vi "base color selection_N.vi"(10 "path":string="000.csv", 11 "Sample Sequence":string="GATGATGATGATGATGAT") -> (2 "element":string, 3 "Base All Composition":T1(array[cluster]))   [LabVIEW 2018]
panel:
  out "error out":errorcluster
  in  "error in":errorcluster
  out "Base C":string[](array[string])
  out "Base Composition":string[](array[string])
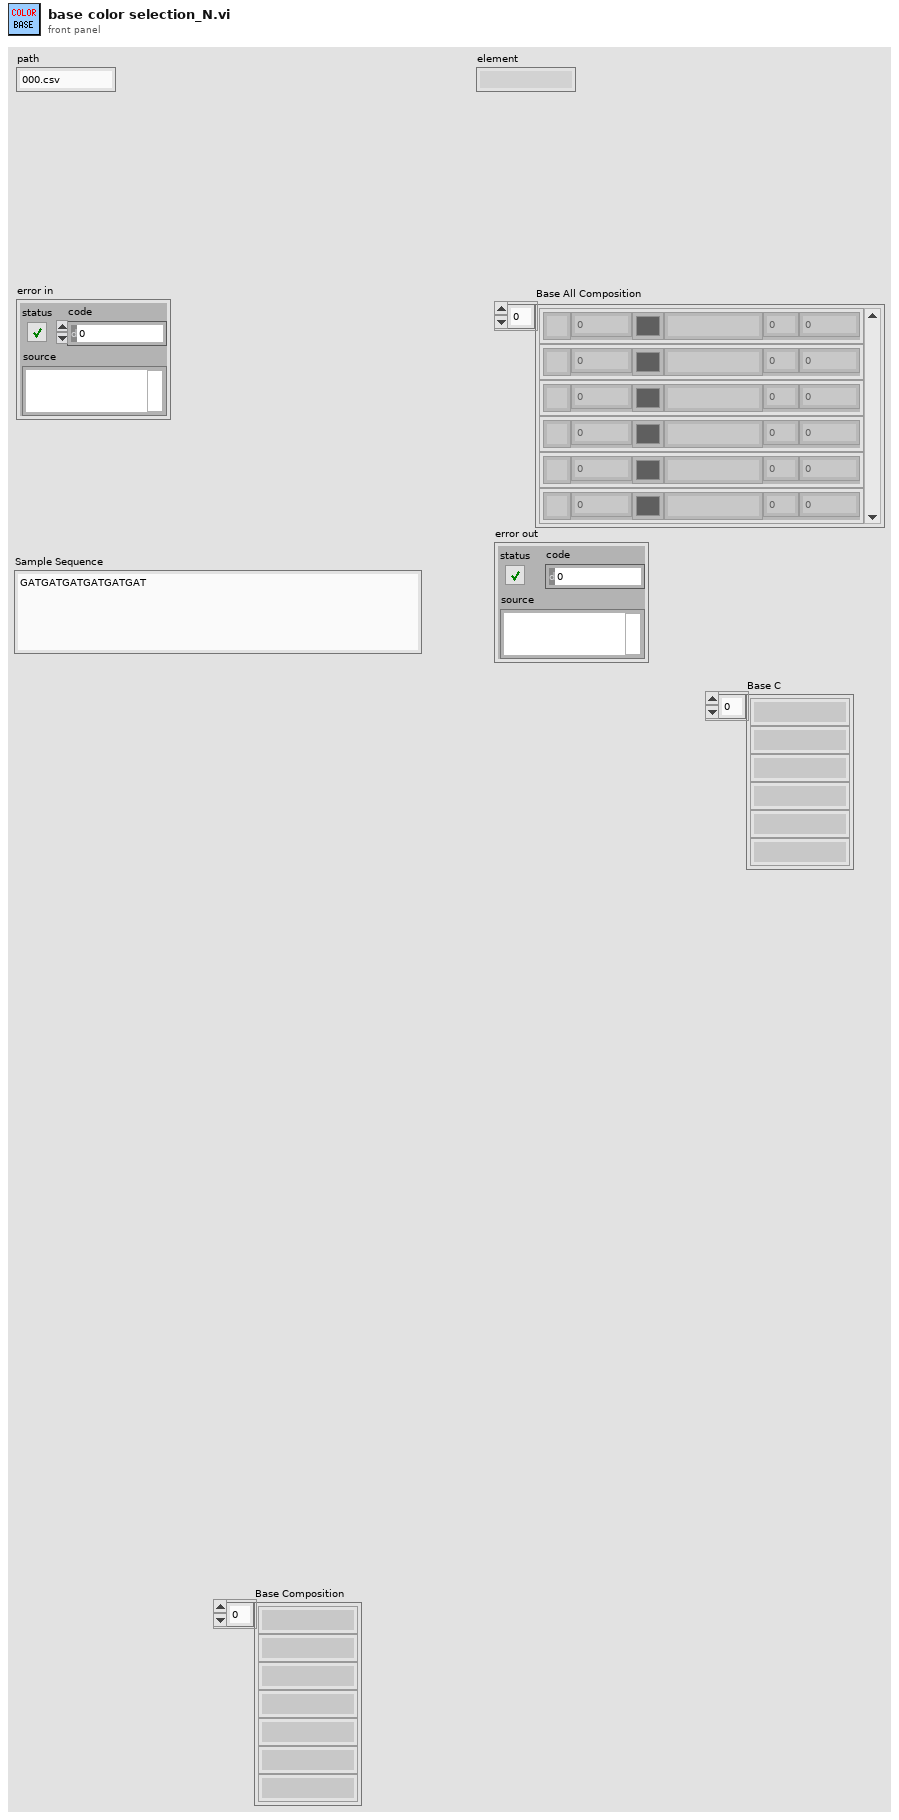
[diagram p1: front panel]
types:
  T1 = cluster{"Name":string, "Value":dbl, "Color":u32, "Name 2":string, "Value 2":dbl, "Value 3":dbl}[]
  T2 = cluster{"Name":string, "Value":dbl, "Color":u32, "Name 2":string, "Value 2":dbl, "Value 3":dbl}
  T3 = cluster{"Base Species IDX":i32, "Item":cluster{"Name":string, "Value":dbl, "Color":u32, "Name 2":string, "Value 2":dbl, "Value 3":dbl}}
  T4 = cluster{"Base Species IDX":i32, "Item":cluster{"Name":string, "Value":dbl, "Color":u32, "Name 2":string, "Value 2":dbl, "Value 3":dbl}}[]
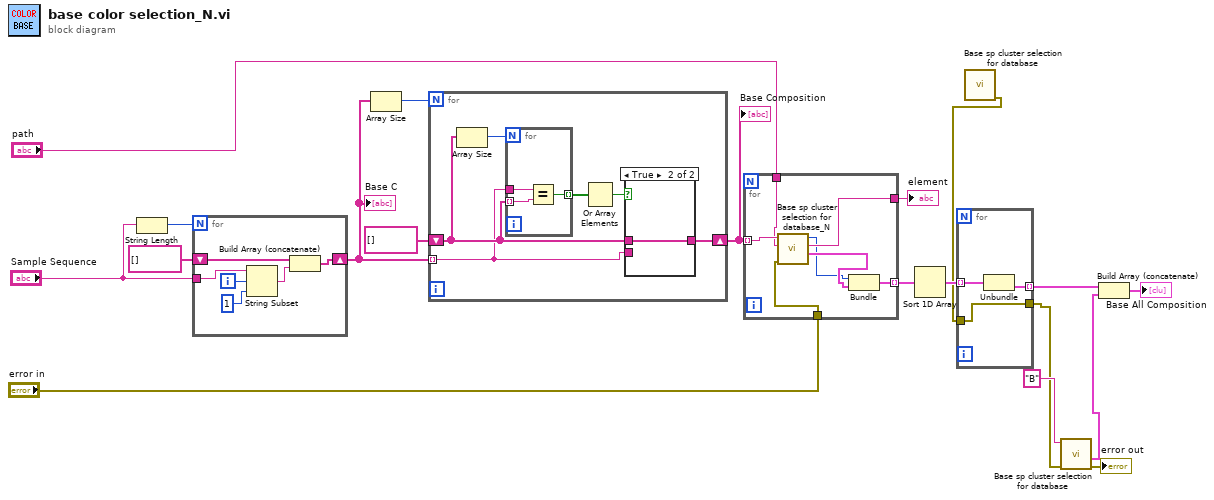
[diagram p0: block diagram]
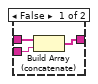
[diagram p2: hidden frame]
diagram:
  n1 = String Length(string="Sample Sequence") -> (length=w19:i32)
  n2 = for {
    N: w19 -> [_]
    tunnel: "Sample Sequence" -> [w23]
    shift-right: [w22] -> w14
    shift-left: string[] [] -> [w21]
    i -> [w24]
    n3 = String Subset(string=w23, offset (0)=w24, length (rest)=1 ("長さ（残り）")) -> (substring=w20:string)
    n4 = Build Array (concatenate)(w21, w20) -> (w22:string[])
  }
  "Base C" <- w14
  n5 = Array Size(array=w14) -> (size(s)=w16:i32)
  n6 = for {
    N: w16 -> [_]
    tunnel: w14 -> [w28] mode=indexing
    shift-right: [w31] -> w11
    shift-left: string[] [] -> [w29]
    n7 = Array Size(array=w29) -> (size(s)=w30:i32)
    n8 = for {
      N: w30 -> [_]
      tunnel: w29 -> [w38] mode=indexing
      tunnel: w28 -> [w37]
      tunnel: [w36] -> w27 mode=indexing
      n9 = Equal?(x=w37, y=w38) -> (x = y?=w36:bool)
    }
    n10 = Or Array Elements(Boolean array=w27) -> (logical OR=w26:bool)
    n11 = case shown="True" w26 {
      tunnel: [w34 w35] -> w31
      tunnel: w29 -> [w33 w35]
      tunnel: w28 -> [w32 _]
      frame False {
        n12 = Build Array (concatenate)(w33, w32) -> (w34:string[])
      }
      frame True {
      }
    }
  }
  "Base Composition" <- w11
  n13 = for {
    tunnel: w11 -> [w43] mode=indexing
    tunnel: [w45] -> w13 mode=indexing
    tunnel: "error in" -> [w44]
    tunnel: [w41] -> w3
    tunnel: "path" -> [w39]
    n14 = call "Base sp cluster selection for database_N.vi"("error in"=w44, "path"=w39, "Base"=w43) -> ("Item"=w42:T2, "element"=w41:string, "Base Species IDX"=w40:i32)  [unwired: 5 in, 1 out]
    n15 = Bundle("Base Species IDX"=w40, "Item"=w42) -> (w45:T3)  [unwired: 1 in]
  }
  "element" <- w3
  n16 = Sort 1D Array(array=w13) -> (sorted array=w12:T4)
  n17 = call "Base sp cluster selection for database.vi"() -> ("error out"=w2:errorcluster)  [unwired: 8 in, 3 out]
  n18 = for {
    tunnel: w12 -> [w48] mode=indexing
    tunnel: [w47] -> w10 mode=indexing
    tunnel: [w46] -> w6
    tunnel: w2 -> [w46]
    n19 = Unbundle(w48) -> ("Item"=w47:T2)  [unwired: 1 out]
  }
  n20 = call "Base sp cluster selection for database.vi"("error in"=w6, "Base"="B") -> ("error out"=→"error out":errorcluster, "Item"=w7:T2)  [unwired: 6 in, 2 out]
  n21 = Build Array (concatenate)(w10, w7) -> (→"Base All Composition":T1)
